vi "Feed Manager.vi"() -> ()   [LabVIEW 2014]
doc: "The NIPM Feed Manager provides a GUI to manage feeds for NI Package Manager packages."
uses:
  _support/Feed Manager States.ctl
  _support/Feed Manager State Data.ctl
  _support/Feed Info.ctl
  _support/UI references.ctl
  <vilib>/Utility/miscctls.llb/LVRowAndColumnTypeDef.ctl
  <vilib>/Utility/sysdir.llb/System Directory Type.ctl
  <vilib>/Utility/miscctls.llb/LVRowAndColumnUnsignedTypeDef.ctl
  <vilib>/National Instruments/NIPM API (Beta)/NIPM_API.lvlib
panel:
  in  "Help Button":bool
  out "Package Attributes":string[][](table)
  in  "Refresh":bool
  in  "Packages in Feed":i32(listbox)=-1
  in  "Unpublish Package":bool
  in  "Publish Package":bool
  in  "Configure Feeds":bool
  in  "Feed":string(combo)="Select a Feed..."
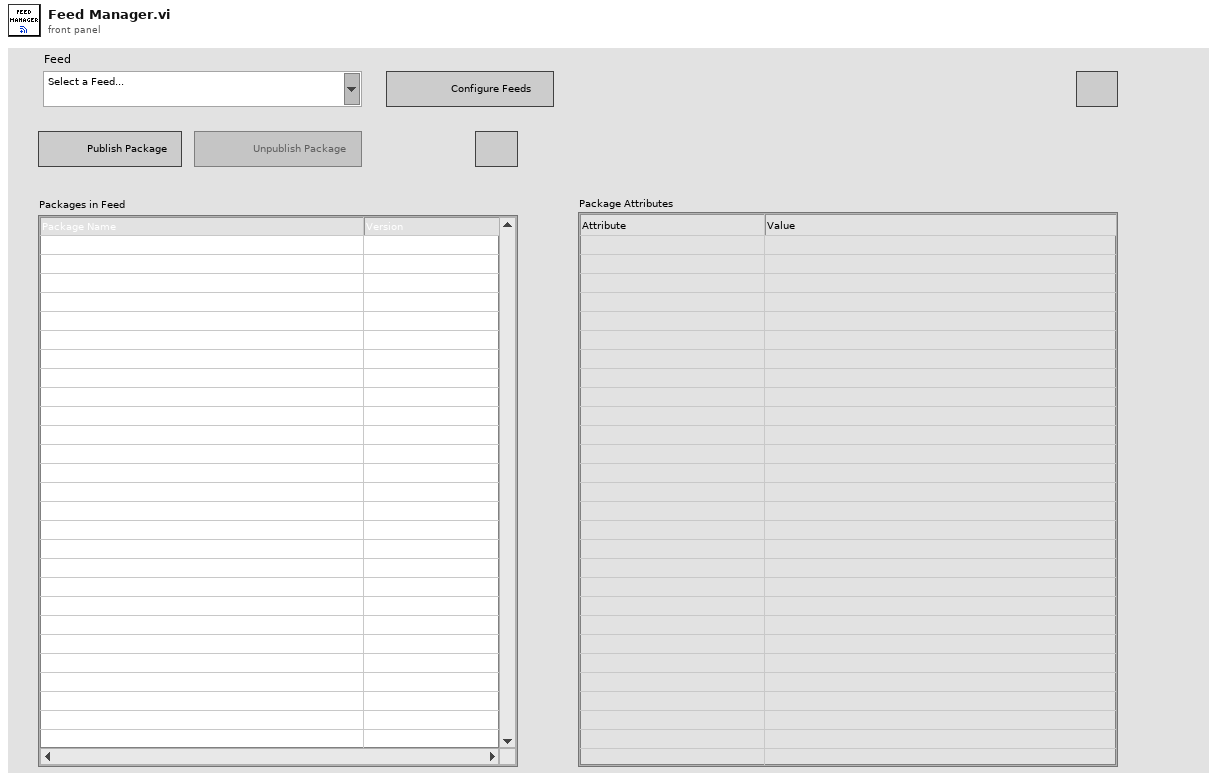
[diagram p1: front panel]
types:
  T1 = typedef "Feed Manager State Data.ctl" = cluster{"Feeds INI Filepath":path, "Current Feed":T2, "Current Row Index":i32, "Managed Feeds":T2[], "Temp Registered Feeds":T2[], "Temp Feed Prefix":string, "Package Relative Filepaths":path[], "UI References":T3}
  T2 = typedef "Feed Info.ctl" = cluster{"Feed Name":string, "Feed Folderpath":string, "Package Destination Folderpath":string}
  T3 = typedef "UI references.ctl" = cluster{"Publish Package":refnum<vi>, "Unpublish Package":refnum<vi>, "Refresh":refnum<vi>, "Packages in Feed":refnum<vi>, "Package Attributes":refnum<vi>}
  T4 = typedef "Feed Manager States.ctl" = enum16{"Initialize", "Wait on Event", "Update Available Feeds", "Configure Feeds", "Update Packages Table", "Update Package Attributes Display", "Publish Package", "Unpublish Package", "Refresh Feed", "Exit"}
  T5 = typedef "LVRowAndColumnTypeDef.ctl" = cluster{"Row":i32, "Column":i32}
  T6 = enum8{"Enabled", "Disabled", "Disabled and Grayed Out"}
  T7 = typedef "LVRowAndColumnUnsignedTypeDef.ctl" = cluster{"Row":u32, "Column":u32}
  T8 = typedef "System Directory Type.ctl" = i32
  T9 = typedef "NIPM_API.lvlib/package attributes.ctl" = cluster{"Package Name":string, "Display name":string, "Version":string, "Display version":string, "Synopsis":string, "Description":string, "Maintainer":string, "Maintainer email address":string, "Category":string, "Homepage":string, "Release notes":string, "Depends":string[], "Recommends":string[], "Suggests":string[], "Conflicts":string[], "Provides":string[], "Replaces":string[], "Supplements":string[], "Enhances":string[], "Product":bool, "User visible":bool, "Installed size (KB)":u64, "Package filesize (bytes)":u64, "Architecture":string, "Agent":string, "MD5Checksum":string}
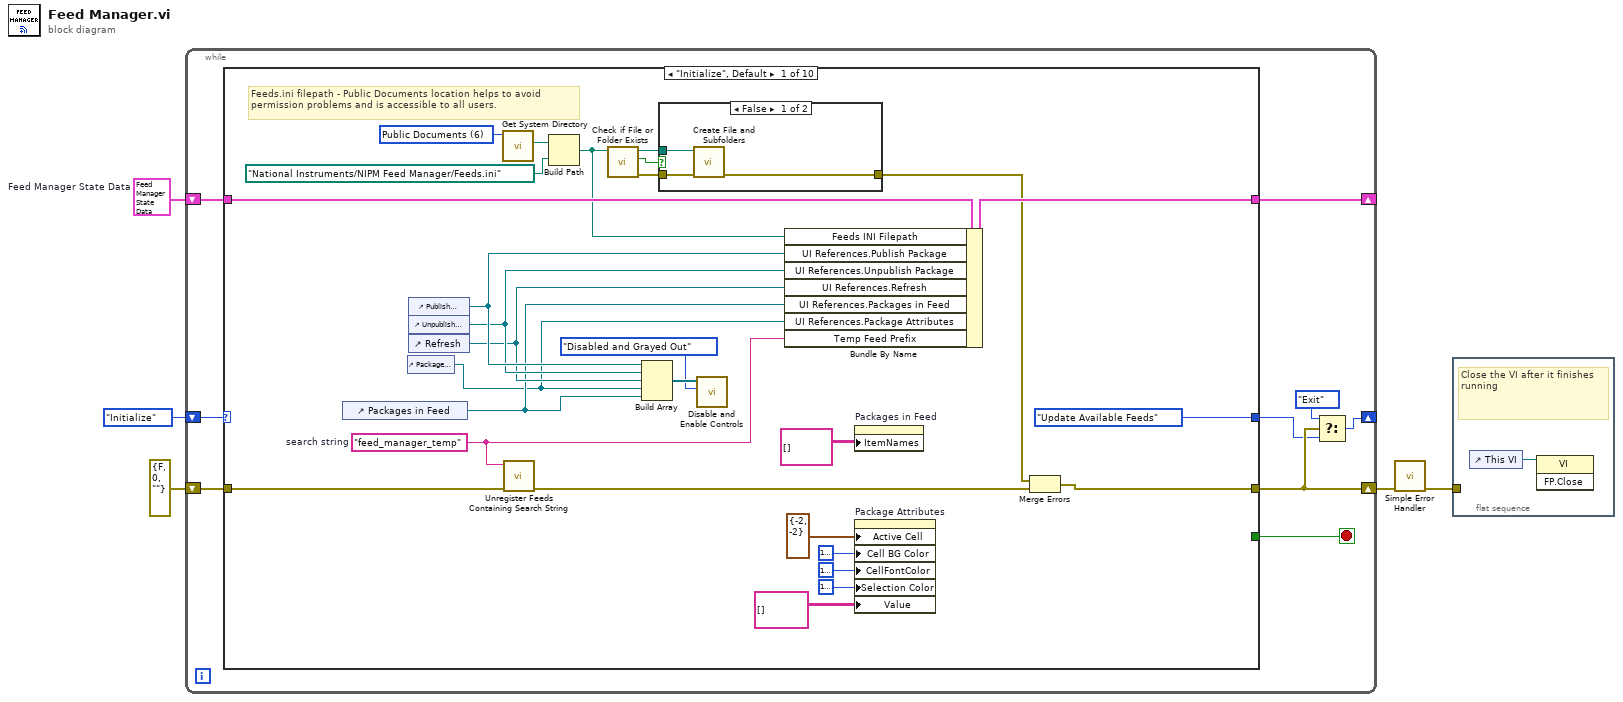
[diagram p0: block diagram]
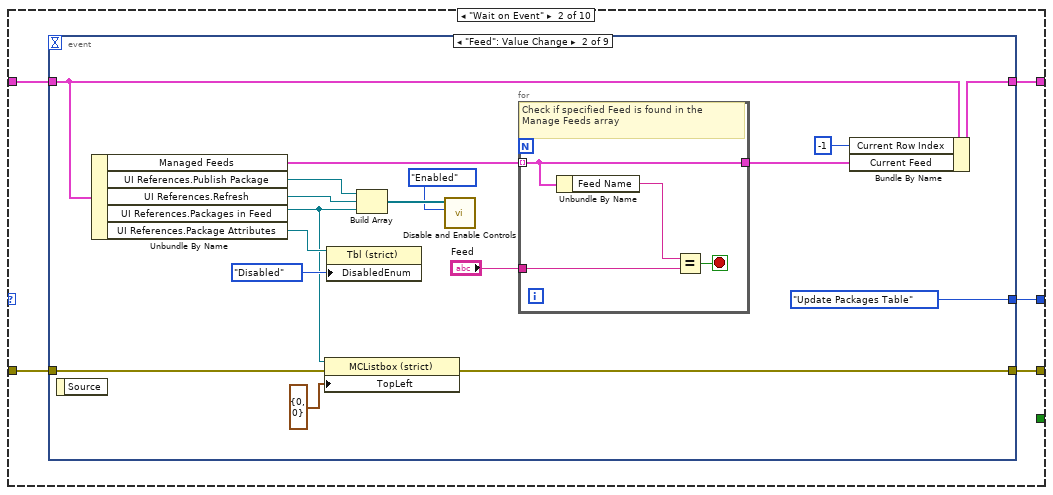
[diagram p3: hidden frame]
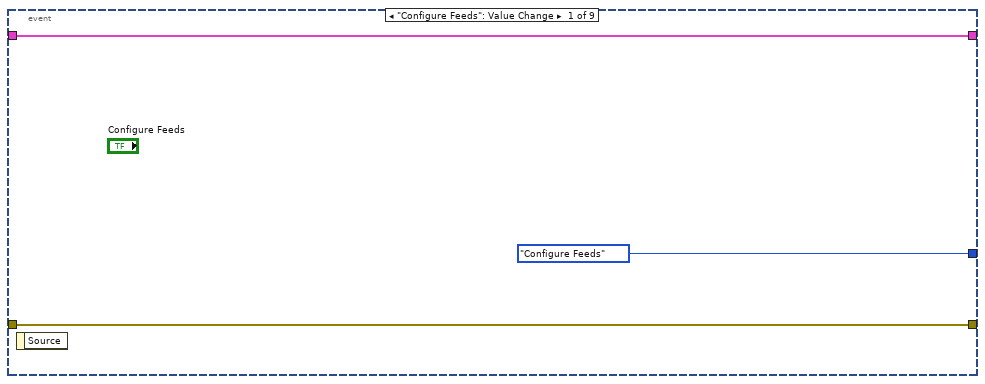
[diagram p4: hidden frame]
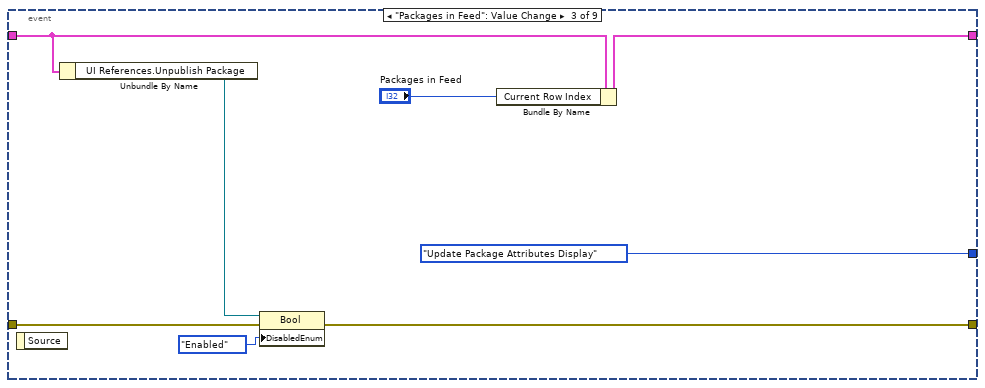
[diagram p5: hidden frame]
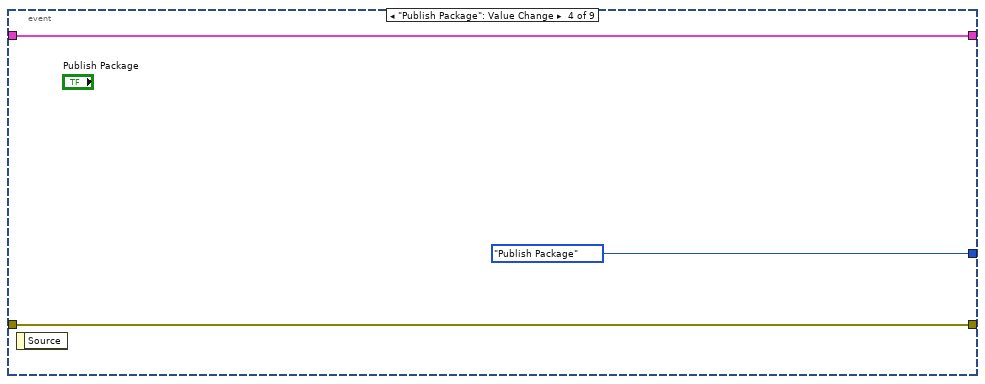
[diagram p6: hidden frame]
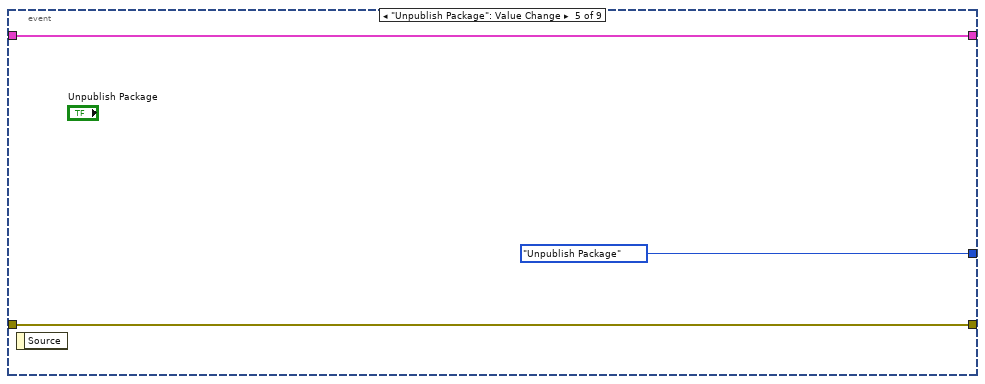
[diagram p7: hidden frame]
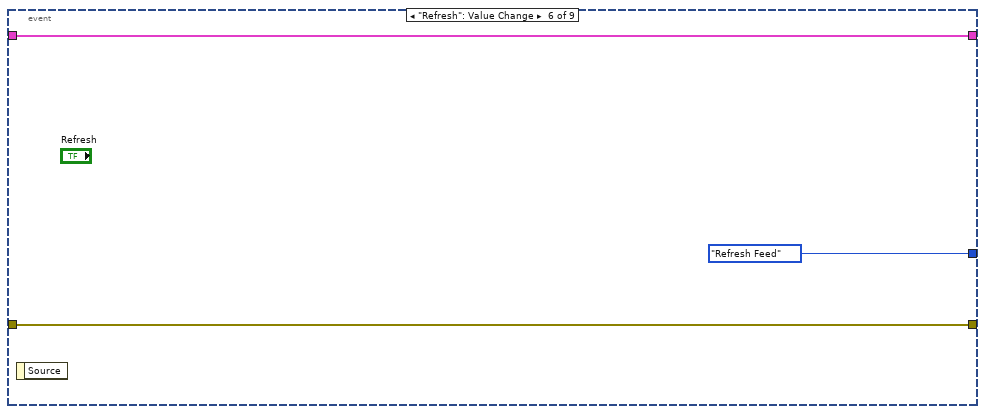
[diagram p8: hidden frame]
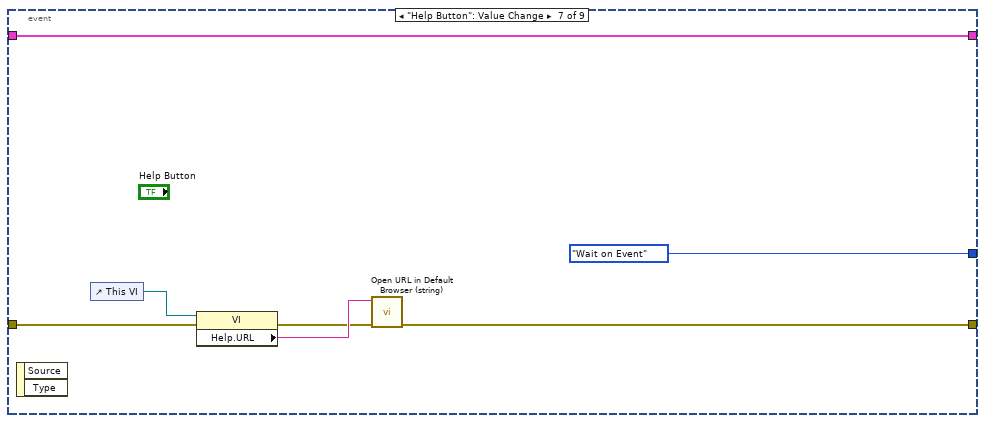
[diagram p9: hidden frame]
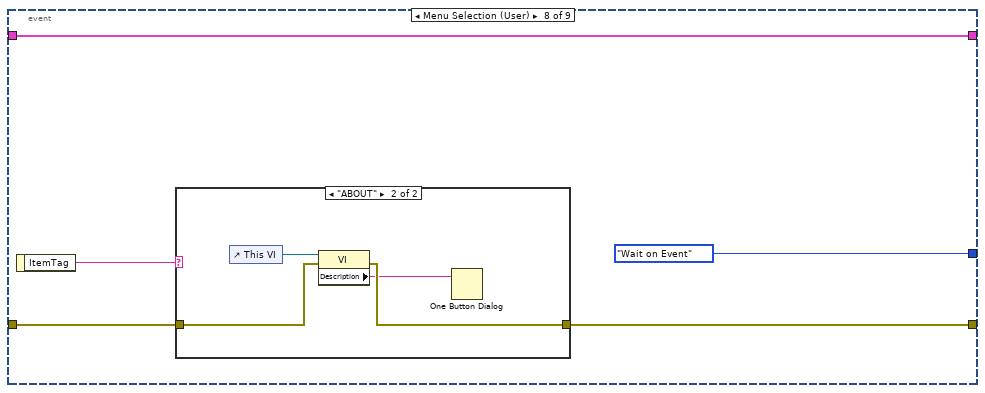
[diagram p10: hidden frame]
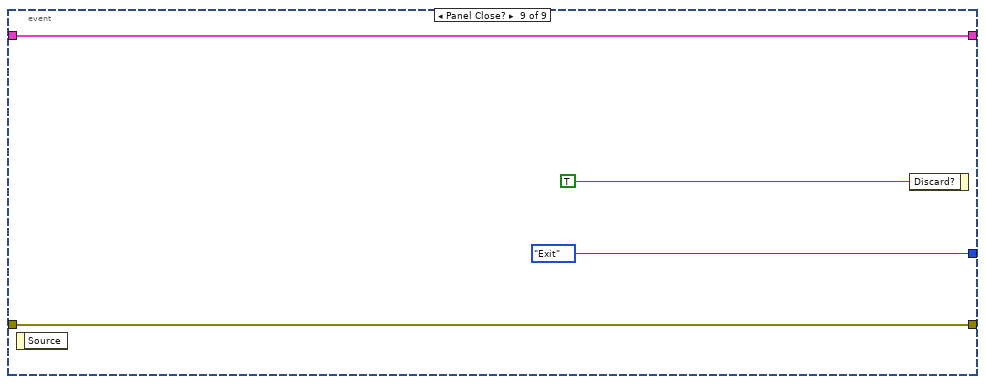
[diagram p12: hidden frame]
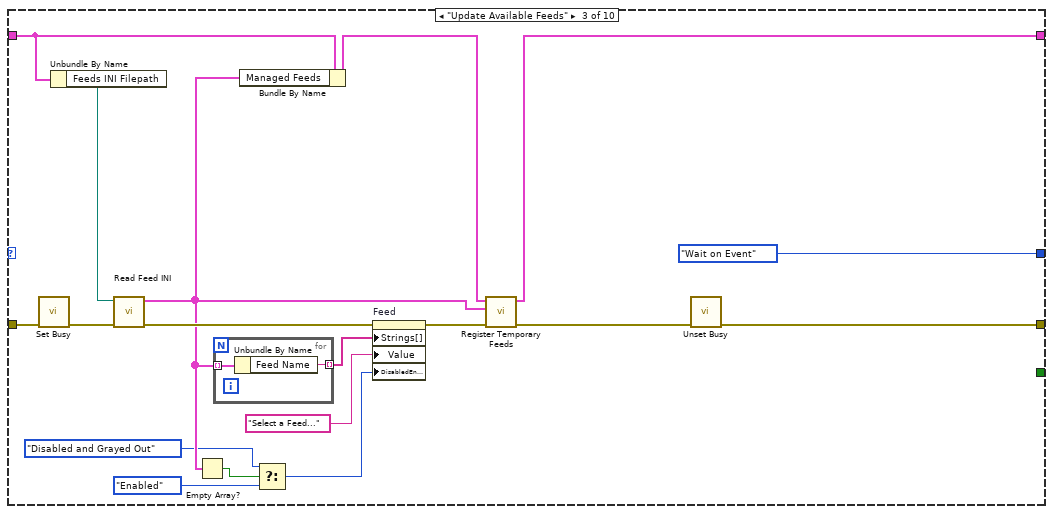
[diagram p13: hidden frame]
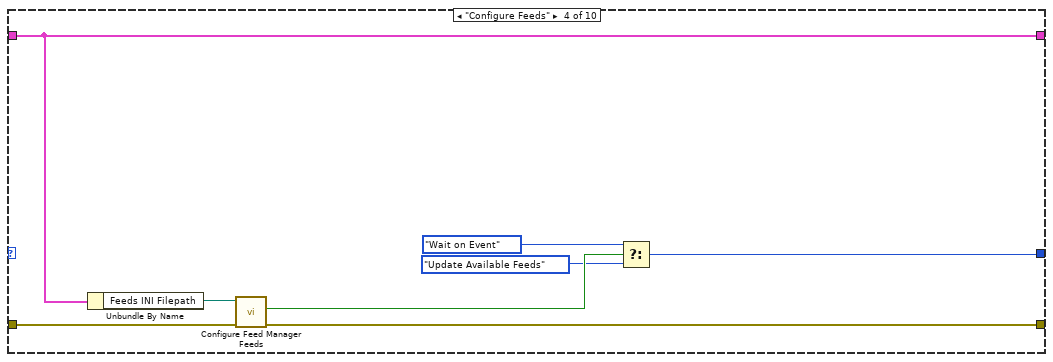
[diagram p14: hidden frame]
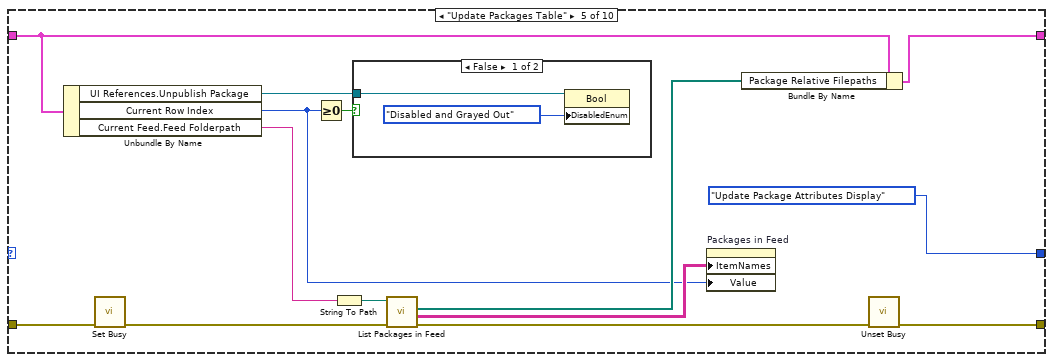
[diagram p15: hidden frame]
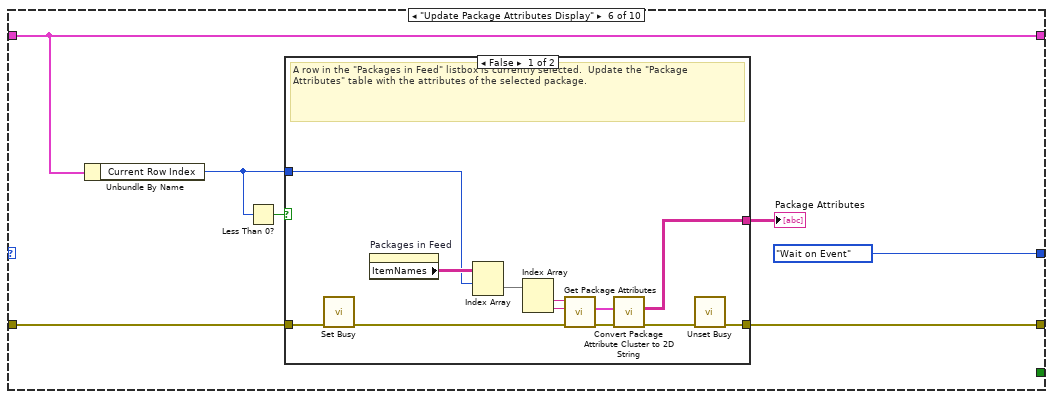
[diagram p17: hidden frame]
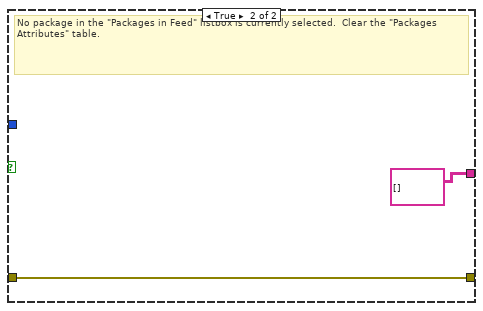
[diagram p18: hidden frame]
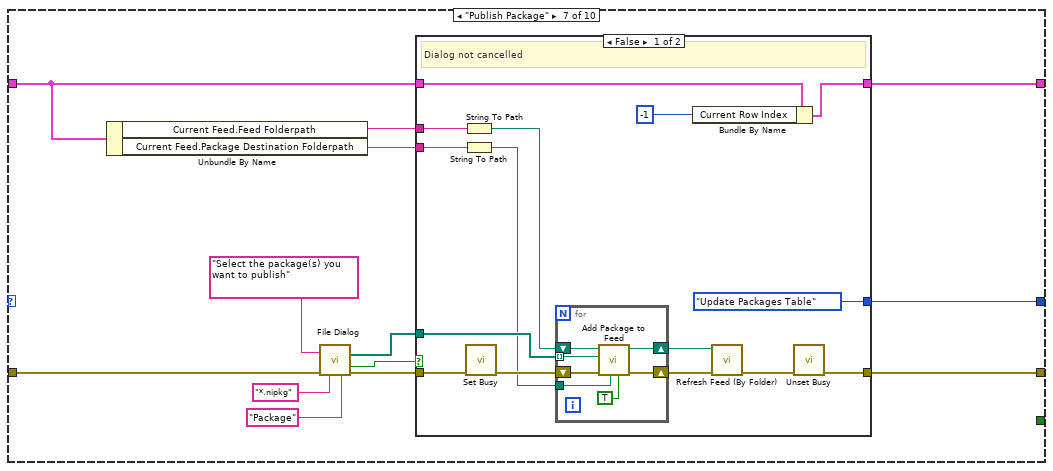
[diagram p19: hidden frame]
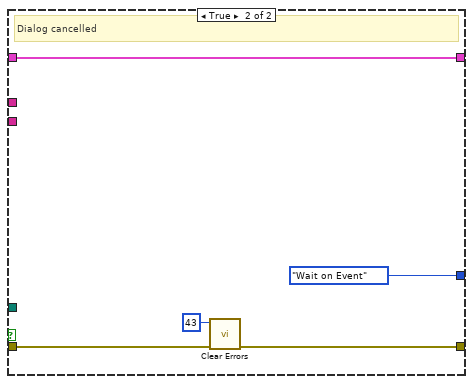
[diagram p20: hidden frame]
diagram:
  w4 = T1 {"Feeds INI Filepath"=path "", "Current Feed"={"Feed Name"="", "Feed Folderpath"="", "Package Destination Folderpath"=""}, "Current Row Index"=-1, "Managed Feeds"=[], "Temp Registered Feeds"=[], "Temp Feed Prefix"="", "Package Relative Filepaths"=[], "UI References"={"Publish Package"=refnum, "Unpublish Package"=refnum, "Refresh"=refnum, "Packages in Feed"=refnum, "Package Attributes"=refnum}}  # Feed Manager State Data
  n1 = while {
    shift-right: [w6] -> _
    shift-left: Feed_Manager_States."Initialize" -> [w14]
    shift-right: [w12] -> _
    shift-left: w4 -> [w13]
    shift-right: [w9] -> w2
    shift-left: errorcluster {"status"=FALSE, "code"=0, "source"=""} ("error in (no error)") -> [w11]
    stop <- w10 stop-if-true
    n2 = case shown="\"Initialize\", Default" w14 {
      tunnel: w13 -> [w42 w50 w124 w135 w153 w162 w182 w232 w239 w252]
      tunnel: [w40 w51 w123 w135 w150 w162 w181 w229 w238 w252] -> w12
      tunnel: [Feed_Manager_States."Update Available Feeds" w47 Feed_Manager_States."Wait on Event" w136 Feed_Manager_States."Update Package Attributes Display" Feed_Manager_States."Wait on Event" w183 Feed_Manager_States."Update Packages Table" Feed_Manager_States."Update Packages Table" Feed_Manager_States."Exit"] -> w8
      tunnel: w11 -> [w25 w49 w131 w138 w152 w164 w186 w233 w242 w255]
      tunnel: [w23 w48 w121 w137 w147 w163 w185 w223 w235 w250] -> w9
      tunnel: [_ _ _ _ _ _ _ _ _ TRUE] -> w10
      frame "Initialize", Default {
        w21 = T8 6 items=["User Home"=0, "User Desktop"=1, "User Documents"=2, "User Application Data"=3, "User Preferences"=4, "User Temporary"=5, "Public Documents"=6, "Public Application Data"=7, "Public Preferences"=8, "Public Cache"=13, "System Core Libraries"=9, "System Installed Libraries"=10, "Application Files"=11, "Boot Volume Root"=12] ("system directory type")
        w26 = "feed_manager_temp"  # search string
        # "Feeds.ini filepath - Public Documents location helps to avoid permission problems and is accessible to all users."
        n3 = control-ref of="Packages in Feed"() -> (w29:refnum<vi>)
        n4 = control-ref of="Package Attributes"() -> (w28:refnum<vi>)
        n5 = control-ref of="Publish Package"() -> (w38:refnum<vi>)
        n6 = control-ref of="Unpublish Package"() -> (w37:refnum<vi>)
        n7 = control-ref of="Refresh"() -> (w34:refnum<vi>)
        n8 = call <vilib>:"Get System Directory.vi"("system directory type"=w21) -> ("system directory"=w20:path)  [unwired: 10 in]
        n9 = call "Unregister Feeds Containing Search String.vi"("error in (no error)"=w25, "search string"=w26) -> ("error out"=w24:errorcluster)  [unwired: 9 in]
        n10 = Build Path(base path=w20, name or relative path=path "National Instruments/NIPM Feed Manager/Feeds.ini") -> (appended path=w18:path)
        n11 = call <vilib>:"Check if File or Folder Exists.vi"("path"=w18) -> ("error out"=w16:errorcluster, "file or folder exists?"=w15:bool, "dup path"=w17:path)  [unwired: 8 in]
        n12 = Build Array(w38, w37, w34, w28, w29) -> (w39:refnum<vi>[])
        n13 = case shown="False" w15 {
          tunnel: [w45 w46] -> w22
          tunnel: w17 -> [w44 _]
          tunnel: w16 -> [w43 w46]
          frame False {
            n14 = call "Create File and Subfolders.vi"("error in (no error)"=w43, "filepath"=w44) -> ("error out"=w45:errorcluster)  [unwired: 9 in]
          }
          frame True {
            # "Feeds.ini file already exists.\nDo nothing."
          }
        }
        n15 = call "Disable and Enable Controls.vi"("Disabled"=T6."Disabled and Grayed Out", "Ctrl Refs"=w39) -> ()  [unwired: 10 in]
        n16 = Bundle By Name(cluster=w42, "Feeds INI Filepath"=w18, "UI References.Publish Package"=w38, "UI References.Unpublish Package"=w37, "UI References.Refresh"=w34, "UI References.Packages in Feed"=w29, "UI References.Package Attributes"=w28, "Temp Feed Prefix"=w26) -> (w40:T1)
        n17 = property on="Packages in Feed" class="MCListbox (strict)"("ItemNames"=string[][] [] ("Item Names")) -> ()  [unwired: 2 in, 2 out]
        n18 = property on="Package Attributes" class="Tbl (strict)"("Active Cell"=T5 {"Row"=-2, "Column"=-2} ("Active Cell:Active Cell"), "Cell BG Color"=u32 16777238, "CellFontColor"=u32 16777222, "Selection Color"=u32 16777224, "Value"=string[][] [] ("Package Attributes")) -> ()  [unwired: 2 in, 2 out]
        n19 = Merge Errors(w22, w24) -> (w23:errorcluster)
      }
      frame "Wait on Event" {
        n20 = event shown="[1] \"Feed\": Value Change" {
          selector: _ -> [_ _ _ _ _ _ _ _ _]
          dyn-events: _ -> [_ _ _ _ _ _ _ _ _]
          timeout: _ -> [_ _ _ _ _ _ _ _ _]
          tunnel: [w54 w70 w82 w86 w89 w91 w99 w104 w113] -> w51
          tunnel: w50 -> [w54 w62 w77 w86 w89 w91 w99 w104 w113]
          tunnel: w49 -> [w53 w57 w80 w85 w88 w90 w94 w102 w112]
          tunnel: [w53 w56 w79 w85 w88 w90 w98 w101 w112] -> w48
          tunnel: [Feed_Manager_States."Configure Feeds" Feed_Manager_States."Update Packages Table" Feed_Manager_States."Update Package Attributes Display" Feed_Manager_States."Publish Package" Feed_Manager_States."Unpublish Package" Feed_Manager_States."Refresh Feed" Feed_Manager_States."Wait on Event" Feed_Manager_States."Wait on Event" Feed_Manager_States."Exit"] -> w47
          event "Configure Feeds": Value Change {
            n21 = event-data() -> ()  [unwired: 1 in, 1 out]
          }
          event "Feed": Value Change {
            n22 = event-data() -> ()  [unwired: 1 in, 1 out]
            n23 = Unbundle By Name(w62) -> ("Managed Feeds"=w61:T2[], "UI References.Publish Package"=w68:refnum<vi>, "UI References.Refresh"=w67:refnum<vi>, "UI References.Packages in Feed"=w58:refnum<vi>, "UI References.Package Attributes"=w64:refnum<vi>)
            n24 = property class="MCListbox (strict)"(reference=w58, error in=w57, "TopLeft"=T7 {"Row"=0, "Column"=0} ("Top Left Visible Cell")) -> (error out=w56:errorcluster)  [unwired: 1 out]
            n25 = property class="Tbl (strict)"(reference=w64, "DisabledEnum"=T6."Disabled" ("Disabled")) -> ()  [unwired: 1 in, 2 out]
            n26 = Build Array(w68, w67, w58) -> (w66:refnum<vi>[])
            n27 = call "Disable and Enable Controls.vi"("Disabled"=T6."Enabled", "Ctrl Refs"=w66) -> ()  [unwired: 10 in]
            n28 = for {
              tunnel: w61 -> [w72] mode=indexing
              tunnel: "Feed" -> [w74]
              tunnel: [w72] -> w59
              stop <- w73 stop-if-true
              # "Check if specified Feed is found in the Manage Feeds array"
              n29 = Unbundle By Name(w72) -> ("Feed Name"=w75:string)
              n30 = Equal?(x=w75, y=w74) -> (x = y?=w73:bool)
            }
            n31 = Bundle By Name(cluster=w62, "Current Row Index"=-1, "Current Feed"=w59) -> (w70:T1)
          }
          event "Packages in Feed": Value Change {
            n32 = event-data() -> ()  [unwired: 1 in, 1 out]
            n33 = Unbundle By Name(w77) -> ("UI References.Unpublish Package"=w78:refnum<vi>)
            n34 = property class="Bool"(reference=w78, error in=w80, "DisabledEnum"=T6."Enabled" ("Disabled")) -> (error out=w79:errorcluster)  [unwired: 1 out]
            n35 = Bundle By Name(cluster=w77, "Current Row Index"="Packages in Feed") -> (w82:T1)
          }
          event "Publish Package": Value Change {
            n36 = event-data() -> ()  [unwired: 1 in, 1 out]
          }
          event "Unpublish Package": Value Change {
            n37 = event-data() -> ()  [unwired: 1 in, 1 out]
          }
          event "Refresh": Value Change {
            n38 = event-data() -> ()  [unwired: 1 in, 1 out]
          }
          event "Help Button": Value Change {
            n39 = event-data() -> ()  [unwired: 1 in, 2 out]
            n40 = control-ref of="This VI"() -> (w96:refnum<vi>)
            n41 = property class="VI"(reference=w96, error in=w94) -> (error out=w93:errorcluster, "Help.URL"=w95:string)  [unwired: 1 out]
            n42 = call <vilib>:"Open URL in Default Browser (string).vi"("error in (no error)"=w93, "URL"=w95) -> ("error out"=w98:errorcluster)  [unwired: 4 in, 1 out]
          }
          event Menu Selection (User) {
            n43 = event-data() -> ("ItemTag"=w103:string)  [unwired: 1 in]
            n44 = case shown="\"ABOUT\"" w103 {
              tunnel: w102 -> [w105 w108]
              tunnel: [w105 w107] -> w101
              frame Default {
              }
              frame "ABOUT" {
                n45 = control-ref of="This VI"() -> (w109:refnum<vi>)
                n46 = property class="VI"(reference=w109, error in=w108) -> (error out=w107:errorcluster, "Description"=w106:string)  [unwired: 1 out]
                n47 = One Button Dialog(message=w106) -> ()  [unwired: 1 in, 1 out]
              }
            }
          }
          event Panel Close? {
            n48 = event-data() -> ()  [unwired: 1 in, 1 out]
            n49 = event-data("Discard?"=TRUE) -> ()  [unwired: 1 in, 1 out]
          }
        }
      }
      frame "Update Available Feeds" {
        n50 = call <vilib>:"Set Busy.vi"("error in (no error)"=w131) -> ("error out"=w122:errorcluster)  [unwired: 9 in, 1 out]
        n51 = Unbundle By Name(w124) -> ("Feeds INI Filepath"=w130:path)
        n52 = call "Read Feed INI.vi"("error in (no error)"=w122, "feeds INI filepath"=w130) -> ("error out"=w129:errorcluster, "feeds"=w118:T2[])  [unwired: 8 in]
        n53 = Empty Array?(array=w118) -> (empty?=w117:bool)
        n54 = for {
          tunnel: w118 -> [w133] mode=indexing
          tunnel: [w132] -> w120 mode=indexing
          n55 = Unbundle By Name(w133) -> ("Feed Name"=w132:string)
        }
        n56 = Bundle By Name(cluster=w124, "Managed Feeds"=w118) -> (w119:T1)
        n57 = Select(t=T6."Disabled and Grayed Out" ("Disabled"), s=w117, f=T6."Enabled" ("Disabled")) -> (s? t:f=w114:T6)
        n58 = property on="Feed" class="CmbBox"(error in=w129, "Strings[]"=w120, "Value"="Select a Feed...", "DisabledEnum"=w114) -> (error out=w128:errorcluster)  [unwired: 1 in, 1 out]
        n59 = call "Register Temporary Feeds.vi"("error in (no error)"=w128, "Feeds"=w118, "Feed Manager State Data in"=w119) -> ("error out"=w125:errorcluster, "Feed Manager State Data out"=w123:T1)  [unwired: 7 in]
        n60 = call <vilib>:"Unset Busy.vi"("error in (no error)"=w125) -> ("error out"=w121:errorcluster)  [unwired: 10 in]
      }
      frame "Configure Feeds" {
        n61 = Unbundle By Name(w135) -> ("Feeds INI Filepath"=w134:path)
        n62 = call "Configure Feed Manager Feeds.vi"("error in (no error)"=w138, "feeds INI Filepath"=w134) -> ("error out"=w137:errorcluster, "cancelled"=w141:bool)  [unwired: 8 in]
        n63 = Select(t=Feed_Manager_States."Wait on Event", s=w141, f=Feed_Manager_States."Update Available Feeds") -> (s? t:f=w136:T4)
      }
      frame "Update Packages Table" {
        n64 = Unbundle By Name(w153) -> ("UI References.Unpublish Package"=w143:refnum<vi>, "Current Row Index"=w146:i32, "Current Feed.Feed Folderpath"=w145:string)
        n65 = call <vilib>:"Set Busy.vi"("error in (no error)"=w152) -> ("error out"=w148:errorcluster)  [unwired: 9 in, 1 out]
        n66 = Greater Or Equal To 0?(x=w146) -> (x >= 0?=w144:bool)
        n67 = String To Path(string=w145) -> (path=w142:path)
        n68 = case shown="False" w144 {
          tunnel: w143 -> [w156 _]
          frame False {
            n69 = property class="Bool"(reference=w156, "DisabledEnum"=T6."Disabled and Grayed Out" ("Disabled")) -> ()  [unwired: 1 in, 2 out]
          }
          frame True {
          }
        }
        n70 = call <vilib>:"List Packages in Feed.vi"("error in"=w148, "feed folderpath in"=w142) -> ("error out"=w154:errorcluster, "package names and versions"=w155:string[][], "package relative filepaths"=w149:path[])  [unwired: 6 in, 1 out]
        n71 = property on="Packages in Feed" class="MCListbox (strict)"("ItemNames"=w155, "Value"=w146) -> ()  [unwired: 2 in, 2 out]
        n72 = Bundle By Name(cluster=w153, "Package Relative Filepaths"=w149) -> (w150:T1)
        n73 = call <vilib>:"Unset Busy.vi"("error in (no error)"=w154) -> ("error out"=w147:errorcluster)  [unwired: 10 in]
      }
      frame "Update Package Attributes Display" {
        n74 = Unbundle By Name(w162) -> ("Current Row Index"=w160:i32)
        n75 = Less Than 0?(x=w160) -> (x < 0?=w159:bool)
        n76 = case shown="False" w159 {
          tunnel: w164 -> [w172 w178]
          tunnel: [w165 w178] -> w163
          tunnel: w160 -> [w170 _]
          tunnel: [w167 string[][] [] ("package attributes (2D string)")] -> w158
          frame False {
            # "A row in the \"Packages in Feed\" listbox is currently selected.  Update the \"Package Attributes\" table with the attributes of the selected package."
            n77 = call <vilib>:"Set Busy.vi"("error in (no error)"=w172) -> ("error out"=w166:errorcluster)  [unwired: 9 in, 1 out]
            n78 = property on="Packages in Feed" class="MCListbox (strict)"() -> ("ItemNames"=w173:string[][])  [unwired: 2 in, 2 out]
            n79 = Index Array(array=w173, index (row)=w170) -> (element=w174:string[])  [unwired: 1 in]
            n80 = Index Array(array=w174) -> (element #1=w175:string, element #2=w176:string)  [unwired: 2 in]
            n81 = call <vilib>:"Get Package Attributes.vi"("error in"=w166, "version"=w176, "package name"=w175) -> ("error out"=w171:errorcluster, "package attributes"=w168:T9)  [unwired: 5 in, 2 out]
            n82 = call <vilib>:"Convert Package Attribute Cluster to 2D String.vi"("error in (no error)"=w171, "package attributes (cluster)"=w168) -> ("error out"=w169:errorcluster, "package attributes (2D string)"=w167:string[][])  [unwired: 8 in]
            n83 = call <vilib>:"Unset Busy.vi"("error in (no error)"=w169) -> ("error out"=w165:errorcluster)  [unwired: 10 in]
          }
          frame True {
            # "No package in the \"Packages in Feed\" listbox is currently selected.  Clear the \"Packages Attributes\" table."
          }
        }
        "Package Attributes" <- w158
      }
      frame "Publish Package" {
        n84 = Unbundle By Name(w182) -> ("Current Feed.Feed Folderpath"=w184:string, "Current Feed.Package Destination Folderpath"=w180:string)
        n85 = call "File Dialog"("prompt"="Select the package(s) you want to publish", "error in"=w186, "pattern (all files)"="*.nipkg", "pattern label"="Package") -> ("selected paths"=w179:path[], "cancelled"=w191:bool, "error out"=w190:errorcluster)  [unwired: 8 in, 1 out]
        n86 = case shown="False" w191 {
          tunnel: w179 -> [w206 _]
          tunnel: w184 -> [w204 _]
          tunnel: w190 -> [w205 w217]
          tunnel: [w200 w215] -> w185
          tunnel: [Feed_Manager_States."Update Packages Table" Feed_Manager_States."Wait on Event"] -> w183
          tunnel: w182 -> [w196 w214]
          tunnel: [w195 w214] -> w181
          tunnel: w180 -> [w194 _]
          frame False {
            # "Dialog not cancelled"
            n87 = String To Path(string=w204) -> (path=w193:path)
            n88 = String To Path(string=w194) -> (path=w192:path)
            n89 = call <vilib>:"Set Busy.vi"("error in (no error)"=w205) -> ("error out"=w201:errorcluster)  [unwired: 9 in, 1 out]
            n90 = for {
              tunnel: w206 -> [w213] mode=indexing
              tunnel: w192 -> [w207]
              shift-right: [w212] -> w202
              shift-left: w201 -> [w211]
              shift-right: [w210] -> w198
              shift-left: w193 -> [w208]
              n91 = call <vilib>:"Add Package to Feed.vi"("create new package destination folderpath if none exists (F)"=TRUE, "package destination folderpath"=w207, "error in"=w211, "package source filepath"=w213, "feed folderpath in"=w208) -> ("error out"=w212:errorcluster, "feed folderpath out"=w210:path)  [unwired: 4 in, 1 out]
            }
            n92 = Bundle By Name(cluster=w196, "Current Row Index"=-1) -> (w195:T1)
            n93 = call <vilib>:"Refresh Feed (By Folder).vi"("error in"=w202, "feed folderpath in"=w198) -> ("error out"=w199:errorcluster)  [unwired: 8 in, 1 out]
            n94 = call <vilib>:"Unset Busy.vi"("error in (no error)"=w199) -> ("error out"=w200:errorcluster)  [unwired: 10 in]
          }
          frame True {
            # "Dialog cancelled"
            n95 = call <vilib>:"Clear Errors.vi"("error in (no error)"=w217, "specific error code to clear (0: all)"=43) -> ("error out"=w215:errorcluster)  [unwired: 4 in, 1 out]
          }
        }
      }
      frame "Unpublish Package" {
        n96 = Unbundle By Name(w232) -> ("Current Feed.Feed Folderpath"=w231:string, "Package Relative Filepaths"=w226:path[], "Current Row Index"=w225:i32)
        n97 = call <vilib>:"Set Busy.vi"("error in (no error)"=w233) -> ("error out"=w221:errorcluster)  [unwired: 9 in, 1 out]
        n98 = Index Array(array=w226, index=w225) -> (element=w234:path)
        n99 = String To Path(string=w231) -> (path=w219:path)
        n100 = Strip Path(path=w234) -> (name=w224:string)  [unwired: 1 out]
        n101 = call <vilib>:"Remove Package from Feed.vi"("error in"=w221, "package filename"=w224, "feed folderpath in"=w219) -> ("error out"=w227:errorcluster, "removed package filepath"=w222:path)  [unwired: 5 in, 2 out]
        n102 = call <vilib>:"Unset Busy.vi"("error in (no error)"=w227) -> ("error out"=w220:errorcluster)  [unwired: 10 in]
        n103 = call "Remove Package Dialog.vi"("error in (no error)"=w220, "removed package filepath"=w222) -> ("error out"=w223:errorcluster)  [unwired: 9 in]
        n104 = Bundle By Name(cluster=w232, "Current Row Index"=-1) -> (w229:T1)
      }
      frame "Refresh Feed" {
        n105 = call <vilib>:"Set Busy.vi"("error in (no error)"=w242) -> ("error out"=w236:errorcluster)  [unwired: 9 in, 1 out]
        n106 = Unbundle By Name(w239) -> ("Feeds INI Filepath"=w245:path)
        n107 = call "Read Feed INI.vi"("error in (no error)"=w236, "feeds INI filepath"=w245) -> ("error out"=w243:errorcluster, "feeds"=w244:T2[])  [unwired: 8 in]
        n108 = for {
          tunnel: w244 -> [w249] mode=indexing
          shift-right: [w246] -> w241
          shift-left: w243 -> [w247]
          # "Refresh data from all feeds listed in Feeds.ini file"
          n109 = Unbundle By Name(w249) -> ("Feed Folderpath"=w248:string)
          n110 = call <vilib>:"Refresh Feed (By URI).vi"("error in (no error)"=w247, "feed URI in"=w248) -> ("error out"=w246:errorcluster)  [unwired: 8 in, 1 out]
        }
        n111 = Bundle By Name(cluster=w239, "Current Row Index"=-1) -> (w238:T1)
        n112 = call <vilib>:"Unset Busy.vi"("error in (no error)"=w241) -> ("error out"=w235:errorcluster)  [unwired: 10 in]
      }
      frame "Exit" {
        n113 = Unbundle By Name(w252) -> ("Temp Registered Feeds"=w251:T2[])
        n114 = for {
          shift-right: [w258] -> w250
          shift-left: w255 -> [w259]
          tunnel: w251 -> [w257] mode=indexing
          # "Unregister temporarily registered feeds"
          n115 = Unbundle By Name(w257) -> ("Feed Name"=w256:string)
          n116 = call <vilib>:"Unregister Feed.vi"("error in"=w259, "feed name"=w256) -> ("error out"=w258:errorcluster)  [unwired: 8 in, 1 out]
        }
      }
    }
    n117 = Select(t=Feed_Manager_States."Exit", s=w9, f=w8) -> (s? t:f=w6:T4)
  }
  n118 = call <vilib>:"Simple Error Handler.vi"("error in (no error)"=w2) -> ("error out"=w1:errorcluster)  [unwired: 4 in, 4 out]
  n119 = flat-sequence {
    tunnel: w1 -> [_]
    frame #0 {
      # "Close the VI after it finishes running"
      n120 = control-ref of="This VI"() -> (w260:refnum<vi>)
      n121 = invoke class="VI" method="FP.Close"(reference=w260) -> ()  [unwired: 2 in, 3 out]
    }
  }
